vi "N10-H16.vi"(11 "Str_10":string) -> (3 "Str_16":string)   [LabVIEW 2025, in "Procotol_class.lvclass"]
uses:
  Procotol_class.lvclass
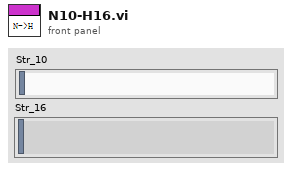
[diagram p1: front panel]
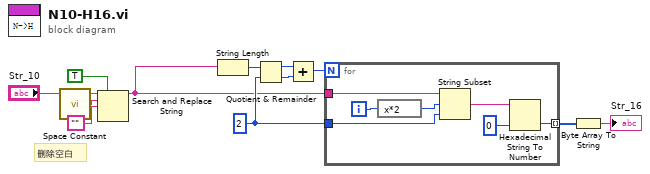
[diagram p0: block diagram]
diagram:
  w4 = 2 ("y")
  # "删除空白"
  n1 = call <vilib>:"Space Constant.vi"() -> ("String"=w11:string)
  n2 = Search and Replace String(replace all?=TRUE ("替换全部？(F)"), input string="Str_10", search string=w11, replace string="") -> (result string=w2:string)  [unwired: 4 in, 3 out]
  n3 = String Length(string=w2) -> (length=w8:i32)
  n4 = Quotient & Remainder(x=w8, y=w4) -> (x-y*floor(x/y)=w7:i32, floor(x/y)=w6:i32)
  n5 = Add(x=w7, y=w6) -> (x+y=w5:i32)
  n6 = for {
    N: w5 -> [_]
    tunnel: w2 -> [w16]
    tunnel: [w17] -> w3 mode=indexing
    tunnel: w4 -> [w14]
    i -> [w19]
    n7 = expression code="x*2"(w19) -> (w15:i32)
    n8 = String Subset(string=w16, offset (0)=w15, length (rest)=w14) -> (substring=w13:string)
    n9 = Hexadecimal String To Number(string=w13, default (0uL)=u8 0 ("默认(0 U32)")) -> (number=w17:u8)  [unwired: 1 in, 1 out]
  }
  n10 = Byte Array To String(unsigned byte array=w3) -> (string=→"Str_16":string)
